vi "Create Error (Code).vi"(4 "timestamp? (True)":bool=TRUE, 5 "is warning? (False)":bool, 6 "error override? (True)":bool=TRUE, 7 "arg. call chain? (False)":bool, 8 "error in (no error)":errorcluster, 9 "error arguments (\"\")":string, 10 "error description (\"\")":string, 11 "error code":i32) -> (0 "error out":errorcluster)   [LabVIEW 2019, in "Error Generation.lvlib"]
doc: "Creates an error with an error error code.\nThis function is similar to original NI \"Error Cluster From Error Code.vi\". Additional functions:\n<b>timestamp?</b>\nadd a current date & time string to the error description.\n<b>error override?</b>\nOverride the error on the input with the error code, despriction & arguments. \n<b>error arguments</b>\nInsert an argument name and data in this format: argument=argument data\nMultiple Arguments can be inserted EOL separated.\nUse arguments, to specify the error more detailled.\n- - -\nCopyright (c) 2023, Merecs Engineering GmbH"
uses:
  Error Generation.lvlib
  Get Argument.vi
  support/Is Error Code.vi
  String to Match Pattern Case Insensitive.vi
  <vilib>/Utility/error.llb/Trim Whitespace.vi
  <vilib>/Utility/error.llb/Check Special Tags.vi
panel:
  # "Connector Pane"
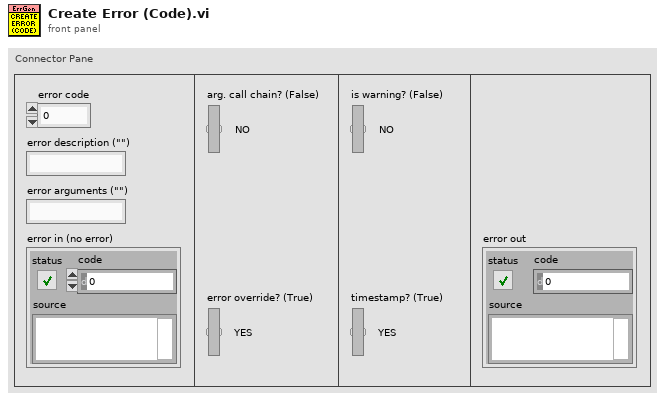
[diagram p1: front panel]
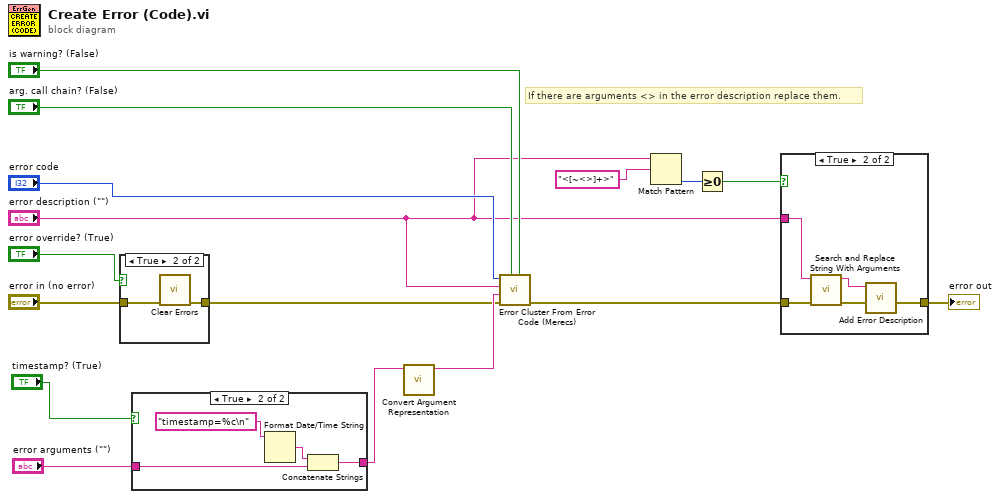
[diagram p0: block diagram]
diagram:
  # "If there are arguments <> in the error description replace them."
  n1 = case shown="True" "error override? (True)" {
    tunnel: "error in (no error)" -> [w17 w19]
    tunnel: [w17 w18] -> w4
    frame False {
    }
    frame True {
      n2 = call <vilib>:"Clear Errors.vi"("error in (no error)"=w19) -> ("error out"=w18:errorcluster)  [unwired: 5 in, 1 out]
    }
  }
  n3 = case shown="True" "timestamp? (True)" {
    tunnel: "error arguments (\"\")" -> [w20 w22]
    tunnel: [w20 w21] -> w2
    frame False {
    }
    frame True {
      n4 = Format Date/Time String(time format string (%c)="timestamp=%c\n") -> (date/time string=w23:string)  [unwired: 2 in]
      n5 = Concatenate Strings(w23, w22) -> (w21:string)
    }
  }
  n6 = call "Convert Argument Representation.vi"("error argument string"=w2) -> ("Formatted Argument"=w11:string)  [unwired: 7 in, 2 out]
  n7 = call "Error Cluster From Error Code (Merecs).vi"("is warning? (False)"="is warning? (False)", "show call chain? (False)"="arg. call chain? (False)", "error in (no error)"=w4, "error arguments (\"\")"=w11, "error description (\"\")"="error description (\"\")", "error code (0)"="error code") -> ("error out"=w1:errorcluster)  [unwired: 3 in]
  n8 = Match Pattern(string="error description (\"\")", regular expression="<[~<>]+>") -> (offset past match=w8:i32)  [unwired: 1 in, 3 out]
  n9 = Greater Or Equal To 0?(x=w8) -> (x >= 0?=w7:bool)
  n10 = case shown="True" w7 {
    tunnel: [w25 w26] -> w5
    tunnel: "error description (\"\")" -> [_ w30]
    tunnel: w1 -> [w25 w29]
    frame False {
    }
    frame True {
      n11 = call "Search and Replace String With Arguments.vi"("error in (no error)"=w29, "String"=w30) -> ("error out"=w27:errorcluster, "Replaced string"=w28:string)  [unwired: 8 in]
      n12 = call "Add Error Description.vi"("error in (no error)"=w27, "error description"=w28) -> ("error out"=w26:errorcluster)  [unwired: 9 in]
    }
  }
  "error out" <- w5
